vi "Current-Voltage-Temperatures.vi"(0 "VISA resource name":refnum<visa-resource-name>, 11 "error in":errorcluster) -> (4 "VISA resource name out":refnum<visa-resource-name>, 6 "Temperatures":dbl[](array[numeric]), 8 "voltage output":dbl, 10 "CURRENT mA":dbl, 15 "error out":errorcluster)   [LabVIEW 2026]
panel:
  out "size(s)":i32
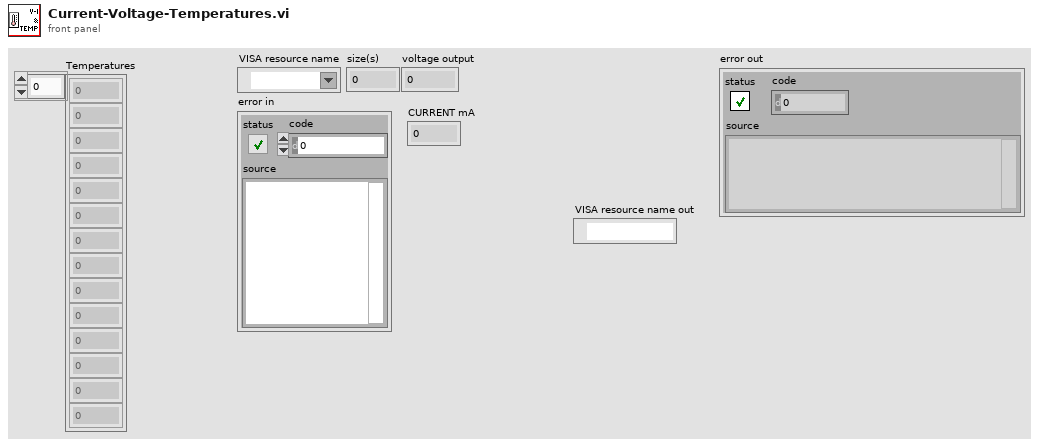
[diagram p1: front panel]
types:
  T1 = cluster{"Mode":enum16{"RTU", "ASCII"}, "Slave Address":u8}
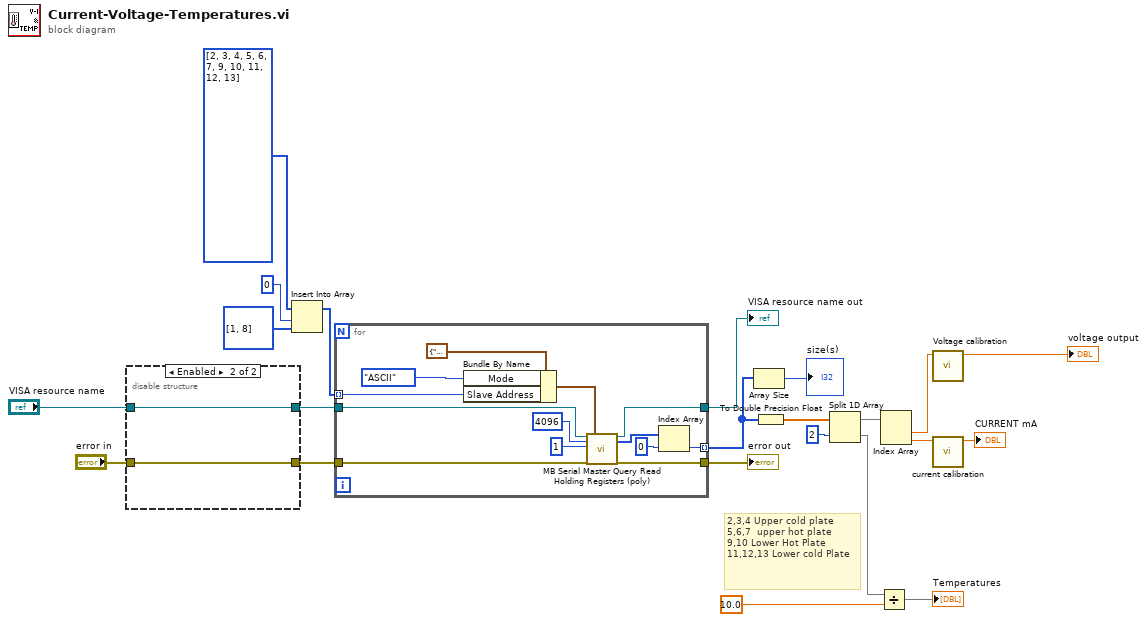
[diagram p0: block diagram]
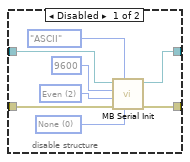
[diagram p2: hidden frame]
diagram:
  # "2,3,4 Upper cold plate\n5,6,7  upper hot plate\n9,10 Lower Hot Plate\n11,12,13 Lower cold Plate"
  n1 = disable-structure shown="Enabled" {
    disable-tunnel: "VISA resource name" -> [w26 w32]
    disable-tunnel: [w25 w31] -> w7
    disable-tunnel: [w24 w32] -> w6
    disable-tunnel: "error in" -> [w23 w31]
    frame Disabled {
      w27 = u16 0 items=["None", "XON/XOFF", "RTS/CTS", "XON/XOFF & RTS/CTS", "DTR/DSR", "XON/XOFF & DTR/DSR"] ("Flow Control")
      w28 = u16 2 items=["None", "Odd", "Even", "Mark", "Space"] ("Parity")
      n2 = call <userlib>:"MB Serial Init.vi"("Flow Control"=w27, "Mode"=enum16{"RTU", "ASCII"}."ASCII", "error in (no error)"=w23, "Parity"=w28, "Baud Rate"=u32 9600, "VISA resource name"=w26) -> ("error out"=w25:errorcluster, "VISA resource name out"=w24:refnum<visa-resource-name>)  [unwired: 4 in]
    }
    frame Enabled {
    }
  }
  n3 = Insert Into Array(array=u8[] [2, 3, 4, 5, 6, 7, 9, 10, 11, 12, 13] ("unit ID"), index=0, new element=u8[] [1, 8]) -> (w17:u8[])
  n4 = for {
    tunnel: w17 -> [w39] mode=indexing
    tunnel: [w44] -> w11 mode=indexing
    tunnel: w7 -> [w42]
    tunnel: w6 -> [w43]
    tunnel: [w34] -> w16
    tunnel: [w33] -> w10
    n5 = Bundle By Name(cluster=T1 {"Mode"=enum."ASCII", "Slave Address"=0} ("Serial Parameters"), "Mode"=enum16{"RTU", "ASCII"}."ASCII", "Slave Address"=w39) -> (w38:T1)
    n6 = call <userlib>:"MB Serial Master Query Read Holding Registers (poly).vi"("VISA resource name"=w43, "Starting Address"=u16 4096 ("starting address"), "Quantity"=u16 1 ("number of inputs"), "error in"=w42, "Serial Parameters"=w38) -> ("VISA resource name out"=w33:refnum<visa-resource-name>, "Holding Registers"=w35:u16[], "error out"=w34:errorcluster)  [unwired: 11 in, 1 out]
    n7 = Index Array(array=w35, index=0) -> (element=w44:u16)
  }
  "error out" <- w16
  "VISA resource name out" <- w10
  n8 = Array Size(array=w11) -> (size(s)=→"size(s)":i32)
  n9 = To Double Precision Float(number=w11) -> (double precision float=w15:dbl[])
  n10 = Split 1D Array(array=w15, index=2) -> (first subarray=w9:dbl[], second subarray=w13:dbl[])
  n11 = Divide(x=w13, y=10.0 ("register")) -> (x/y=→"Temperatures":dbl[])
  n12 = Index Array(array=w9) -> (element #1=w4:dbl, element #2=w2:dbl)  [unwired: 2 in]
  n13 = call "Voltage calibration.vi"("INPUT VOLTAGE"=w4) -> ("voltage output"=→"voltage output":dbl)  [unwired: 10 in]
  n14 = call "current calibration.vi"("Current"=w2) -> ("CURRENT mA"=→"CURRENT mA":dbl)  [unwired: 10 in]
